vi "GetClassNameArray.vi"(8 "error in (no error)":errorcluster, 10 "ClassName Cache":refnum<data-value>, 11 "LabVIEW Object in":refnum<class>) -> (0 "error out":errorcluster, 3 "Class (child,parent)":T1[](array[typedef]))   [LabVIEW 2020, in "BlueSerialization.lvlib" / "BlueSerializer.lvclass"]
uses:
  BlueSerializer.lvclass
  ClassNameCacheCluster.ctl
  ClassNameCacheMap.ctl
  ClassNameObj.ctl
  GetDescendantType.vi
  LVOOP is Same or Descendant Class Inline.vi
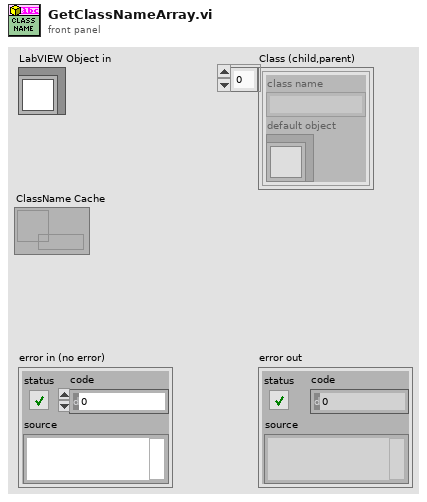
[diagram p1: front panel]
types:
  T1 = typedef "BlueSerialization.lvlib/BlueSerializer.lvclass/ClassNameObj.ctl" = cluster{"class name":string, "default object":refnum<class>}
  T2 = typedef "BlueSerialization.lvlib/BlueSerializer.lvclass/ClassNameCacheCluster.ctl" = cluster{"Classes in memory":refnum<class>[], "Hierarchy Map":T3}
  T3 = typedef "BlueSerialization.lvlib/BlueSerializer.lvclass/ClassNameCacheMap.ctl" = map{string, T1[]}
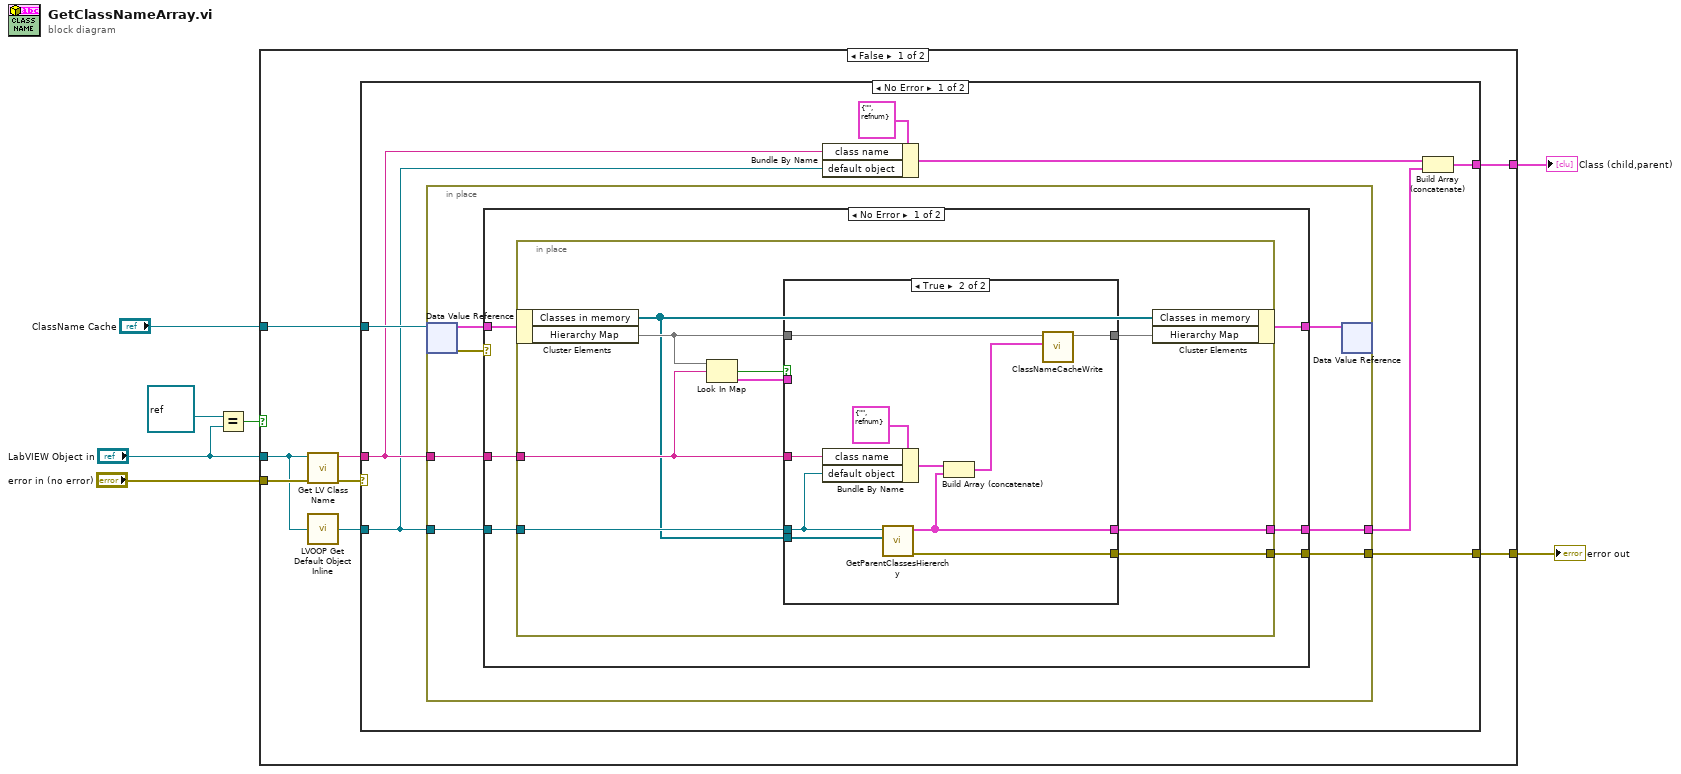
[diagram p0: block diagram]
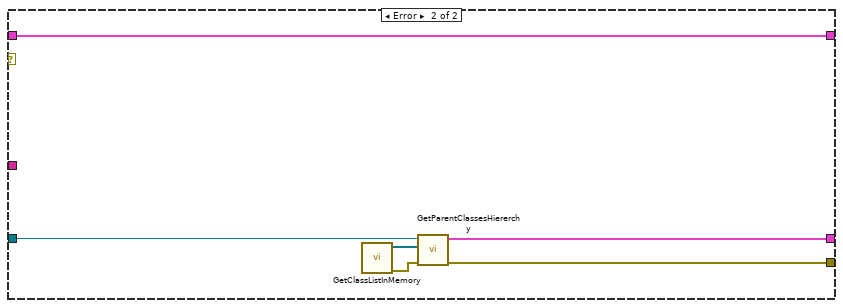
[diagram p3: hidden frame]
diagram:
  n1 = Equal?(x=refnum<class> refnum ("LabVIEW Object"), y="LabVIEW Object in") -> (x = y?=w3:bool)
  n2 = case shown="False" w3 {
    tunnel: "error in (no error)" -> [w14 w65]
    tunnel: [w13 w65] -> w6
    tunnel: [w12 _] -> w1
    tunnel: "LabVIEW Object in" -> [w9 _]
    tunnel: "ClassName Cache" -> [w10 _]
    frame False {
      n3 = call <vilib>:"Get LV Class Name.vi"("error in (no error)"=w14, "object"=w9) -> ("error out"=w11:errorcluster, "class name"=w15:string)  [unwired: 8 in]
      n4 = call "LVOOP Get Default Object Inline.vi"("Object"=w9) -> ("Object Default Instance"=w8:refnum<class>)
      n5 = case shown="No Error" w11 {
        selector: w11 -> [_ w64]
        tunnel: w15 -> [w18 _]
        tunnel: [w20 w64] -> w13
        tunnel: [w22 _] -> w12
        tunnel: w8 -> [w17 _]
        tunnel: w10 -> [w21 _]
        frame No Error {
          n6 = in-place {
            in-place-border: w18 -> [w27]
            in-place-border: [w30] -> w20
            in-place-border: w17 -> [w29]
            in-place-border: [w25] -> w23
            n7 = in-place-dvr #1(w21) -> (w28:T2, w24:errorcluster)
            n8 = case shown="No Error" w24 {
              tunnel: [w36 w62] -> w30
              tunnel: w29 -> [w35 w61]
              tunnel: w28 -> [w32 w63]
              tunnel: w27 -> [w34 _]
              tunnel: [w31 w63] -> w26
              tunnel: [w33 w60] -> w25
              frame No Error {
                n9 = in-place {
                  in-place-border: [w45] -> w36
                  in-place-border: w35 -> [w44]
                  in-place-border: w34 -> [w42]
                  in-place-border: [w40] -> w33
                  n10 = in-place-cluster #2(w32) -> ("Classes in memory"=w37:refnum<class>[], "Hierarchy Map"=w39:T3)
                  n11 = Look In Map(map=w39, key=w42) -> (key not found?=w43:bool, value=w41:T1[])  [unwired: 1 in]
                  n12 = case shown="True" w43 {
                    tunnel: [_ w57] -> w45
                    tunnel: w44 -> [_ w51]
                    tunnel: [w46 w49] -> w40
                    tunnel: w39 -> [w47 w56]
                    tunnel: w42 -> [_ w52]
                    tunnel: [w47 w55] -> w38
                    tunnel: w41 -> [w46 _]
                    tunnel: w37 -> [_ w48]
                    frame False {
                    }
                    frame True {
                      n13 = Bundle By Name(cluster=T1 {"class name"="", "default object"=refnum} ("Cluster"), "class name"=w52, "default object"=w51) -> (w53:T1)
                      n14 = call "GetParentClassesHiererchy.vi"("Classes in memory"=w48, "LabVIEW Object in"=w51) -> ("error out"=w57:errorcluster, "Class (child,parent)"=w49:T1[])  [unwired: 8 in]
                      n15 = Build Array (concatenate)(w53, w49) -> (w50:T1[])
                      n16 = call "ClassNameCacheWrite.vi"("Class (child,parent)"=w50, "Map"=w56) -> ("Map"=w55:T3)  [unwired: 9 in]
                    }
                  }
                  n17 = in-place-cluster #2("Classes in memory"=w37, "Hierarchy Map"=w38) -> (w31:T2)
                }
              }
              frame Error {
                n18 = call "GetClassListInMemory.vi"() -> ("error out"=w59:errorcluster, "Classes in memory"=w58:refnum<class>[])  [unwired: 10 in]
                n19 = call "GetParentClassesHiererchy.vi"("error in (no error)"=w59, "Classes in memory"=w58, "LabVIEW Object in"=w61) -> ("error out"=w62:errorcluster, "Class (child,parent)"=w60:T1[])  [unwired: 7 in]
              }
            }
            n20 = in-place-dvr #1(w26) -> ()  [unwired: 2 out]
          }
          n21 = Bundle By Name(cluster=T1 {"class name"="", "default object"=refnum} ("Cluster"), "class name"=w18, "default object"=w17) -> (w16:T1)
          n22 = Build Array (concatenate)(w16, w23) -> (w22:T1[])
        }
        frame Error {
        }
      }
    }
    frame True {
    }
  }
  "error out" <- w6
  "Class (child,parent)" <- w1
